vi "grafica-de-temperatura.vi"() -> ()   [LabVIEW 2016]
panel:
  out "Lecturas de temperatura":cluster{dbl[], dbl[]}(graph)
  in  "Numero de lecturas":i32
  in  "Tiempo de muestreo (ms)":dbl(knob) scale=0.0..500.0
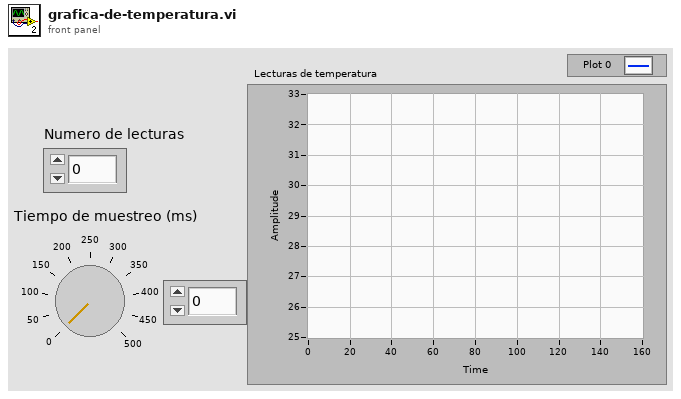
[diagram p1: front panel]
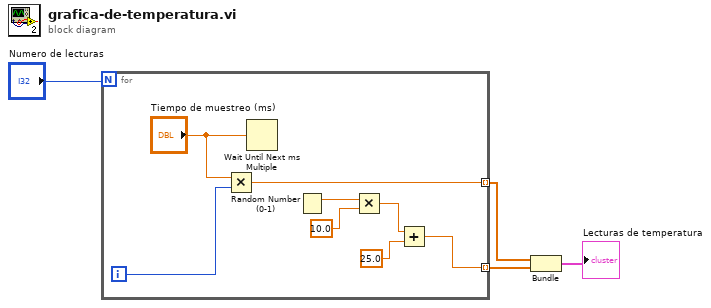
[diagram p0: block diagram]
diagram:
  n1 = for {
    N: "Numero de lecturas" -> [_]
    tunnel: [w8] -> w3 mode=indexing
    tunnel: [w5] -> w2 mode=indexing
    i -> [w6]
    n2 = Multiply(x="Tiempo de muestreo (ms)", y=w6) -> (x*y=w5:dbl)
    n3 = Wait Until Next ms Multiple(millisecond multiple="Tiempo de muestreo (ms)") -> ()  [unwired: 1 out]
    n4 = Random Number (0-1)() -> (number: 0 to 1=w12:dbl)
    n5 = Multiply(x=w12, y=10.0) -> (x*y=w10:dbl)
    n6 = Add(x=w10, y=25.0) -> (x+y=w8:dbl)
  }
  n7 = Bundle(w2, w3) -> (→"Lecturas de temperatura":cluster{dbl[], dbl[]})  [unwired: 1 in]
